vi "myFreqSymm.vi"(6 "基频":u32=50, 10 "注入(1号)端口类型":u8(ring) items=["单相", "三相αβ系", "三相同步系", "三相正负序"], 11 "Freqs in":i32[](array[numeric])=[10, 14, 19, 27, 37, 51, 71, 99, 140, 190, 260, 360, 510, 700, 970, 1400, 1900, 2600, 3600, 5000]) -> (3 "Freqs out":i32[](array[numeric]))   [LabVIEW 2024]
doc: "当待测正负序耦合时：\n1）在原扫频点集基础上扩充密度。\n2）在正频点后面补充一个负轴频点组，用于负序注入的情况。\n当待测同步系耦合时：\n1）从频点组中去掉基波，这是因为dsp端（大概）不能注入直流。"
uses:
  1cbf77b3-6660-4233-b6e1-d199a60284c5.vi
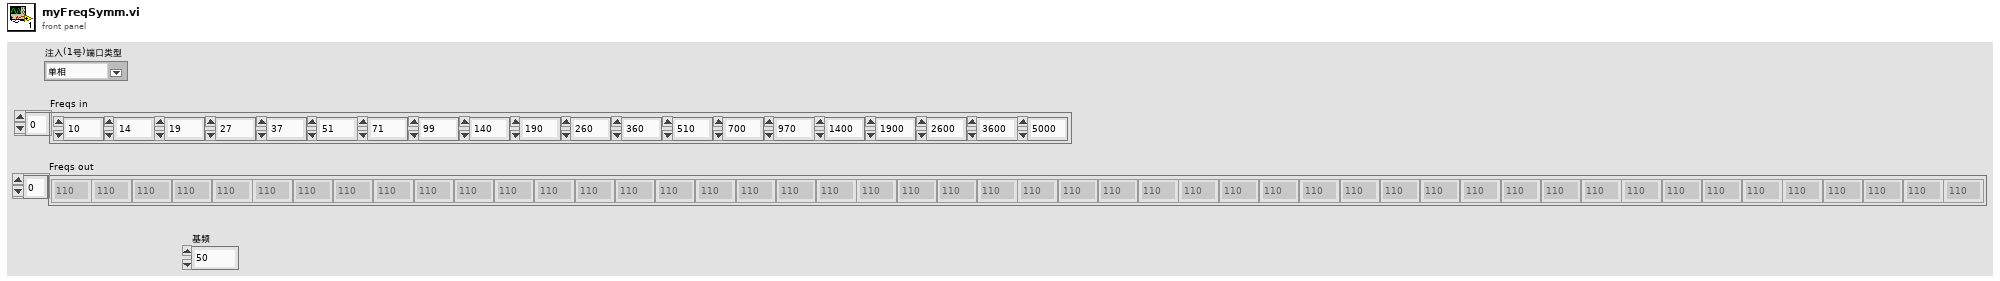
[diagram p1: front panel]
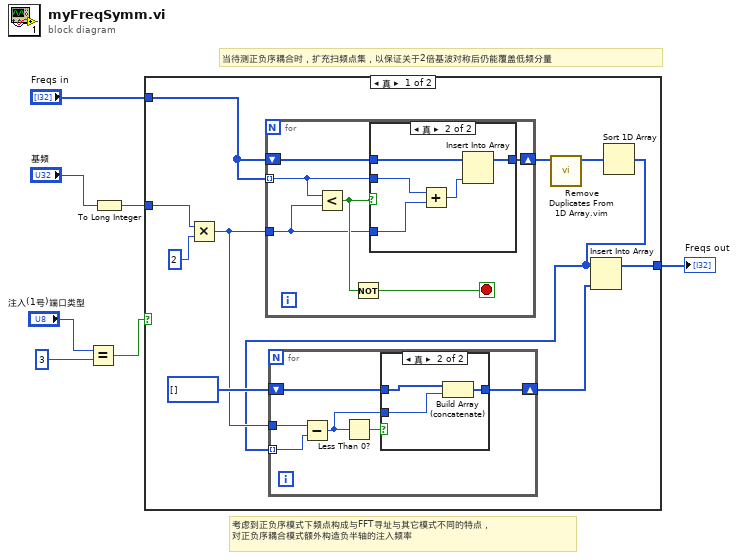
[diagram p0: block diagram]
diagram:
  # "考虑到正负序模式下频点构成与FFT寻址与其它模式不同的特点，\n对正负序耦合模式额外构造负半轴的注入频率"
  # "当待测正负序耦合时，扩充扫频点集，以保证关于2倍基波对称后仍能覆盖低频分量"
  n1 = Equal?(x="注入(1号)端口类型", y=3) -> (x = y?=w1:bool)
  n2 = To Long Integer(number="基频") -> (32bit integer=w6:i32)
  n3 = case shown="真" w1 {
    tunnel: "Freqs in" -> [w15 w40]
    tunnel: [w9 w40] -> w7
    tunnel: w6 -> [w12 _]
    frame True {
      n4 = Multiply(x=w12, y=2) -> (x*y=w11:i32)
      n5 = for {
        tunnel: w15 -> [w29] mode=indexing
        shift-right: [w30] -> w17
        shift-left: w15 -> [w31]
        tunnel: w11 -> [w28]
        stop <- w33 stop-if-true
        n6 = Less?(x=w29, y=w28) -> (x < y?=w32:bool)
        n7 = Not(x=w32) -> (.not. x?=w33:bool)
        n8 = case shown="真" w32 {
          tunnel: w31 -> [w34 w39]
          tunnel: [w34 w38] -> w30
          tunnel: w29 -> [_ w37]
          tunnel: w28 -> [_ w35]
          frame False {
          }
          frame True {
            n9 = Add(x=w37, y=w35) -> (x+y=w36:i32)
            n10 = Insert Into Array(array=w39, new element=w36) -> (w38:i32[])  [unwired: 1 in]
          }
        }
      }
      n11 = call "Remove Duplicates From 1D Array.vim"("array"=w17) -> ("array with duplicates removed"=w16:i32[])  [unwired: 10 in]
      n12 = Sort 1D Array(array=w16) -> (sorted array=w8:i32[])
      n13 = for {
        tunnel: w8 -> [w20] mode=indexing
        shift-right: [w22] -> w10
        shift-left: i32[] [] -> [w23]
        tunnel: w11 -> [w21]
        n14 = Subtract(x=w21, y=w20) -> (x-y=w18:i32)
        n15 = Less Than 0?(x=w18) -> (x < 0?=w19:bool)
        n16 = case shown="真" w19 {
          tunnel: w23 -> [w24 w27]
          tunnel: [w24 w26] -> w22
          tunnel: w18 -> [_ w25]
          frame False {
          }
          frame True {
            n17 = Build Array (concatenate)(w27, w25) -> (w26:i32[])
          }
        }
      }
      n18 = Insert Into Array(array=w8, new element=w10) -> (w9:i32[])  [unwired: 1 in]
    }
    frame False {
    }
  }
  "Freqs out" <- w7
